vi "CPU_IRQ_handle.vi"(11 "registers":T1 {"P" format="%08b"; "PC" format="%04x"; "SP" format="%02x"; "Y" format="%02x"; "X" format="%02x"; "A" format="%02x"}) -> (3 "registers":T1 {"P" format="%08b"; "PC" format="%04x"; "SP" format="%02x"; "Y" format="%02x"; "X" format="%02x"; "A" format="%02x"})   [LabVIEW 2018]
uses:
  CPU_registers.ctl
  memory/CPU_MEM_Char_ROM_RE.vi
  CIA/CIA1/CIA1_glb.vi
  VIC/VIC_glb.vi
  memory/CPU_MEM_RAM.vi
  CPU_Port.vi
  memory/CPU_MEM_RAM_RE.vi
  memory/CPU_MEM_Basic_ROM_RE.vi
  memory/CPU_MEM_references.vi
  memory/CPU_MEM_VIC-II.vi
  memory/CPU_MEM_SID_RE.vi
  memory/CPU_MEM_Color_RE.vi
  memory/CPU_MEM_CIA 1.vi
  memory/CPU_MEM_CIA 2.vi
  memory/CPU_MEM_Kernal_ROM_RE.vi
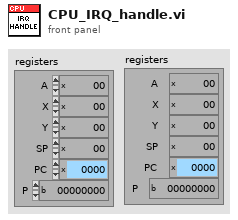
[diagram p1: front panel]
types:
  T1 = typedef "CPU_registers.ctl" = cluster{"A":u8, "X":u8, "Y":u8, "SP":u8, "PC":u16, "P":u8}
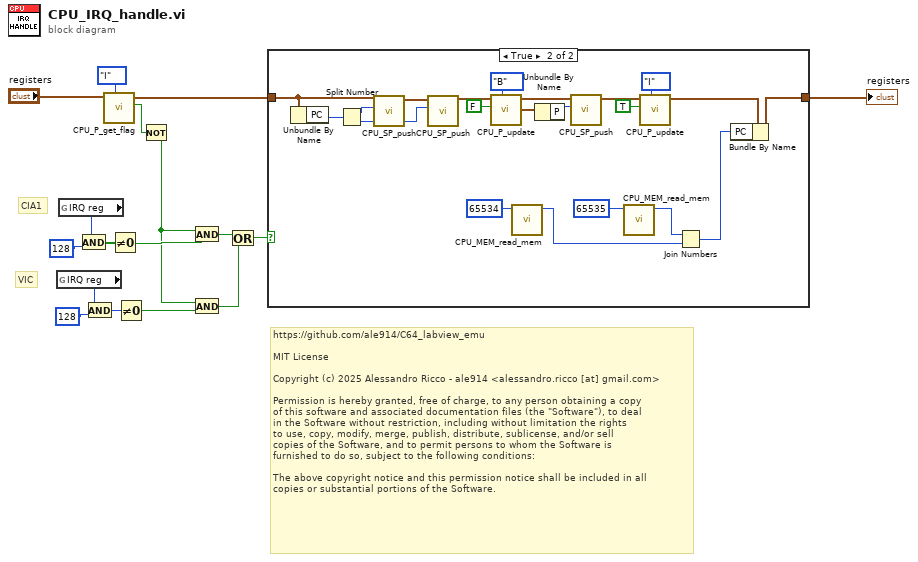
[diagram p0: block diagram]
diagram:
  # "https://github.com/ale914/C64_labview_emu\n\nMIT License\n\nCopyright (c) 2025 Alessandro Ricco - ale914 <alessandro.ricco [at] gmail.com>\n\nPermission is hereby granted, free of charge, to any person obtaining a copy\nof this software and associated documentation files (the \"Software\"), to deal\nin the Software without restriction, including without limitation the rights\nto use, copy, modify, merge, publish, distribute, sublicense, and/or sell\ncopies of the Software, and to permit persons to whom the Software is\nfurnished to do so, subject to the following conditions:\n\nThe above copyright notice and this permission notice shall be included in all\ncopies or substantial portions of the Software."
  # "VIC"
  # "CIA1"
  n1 = global read "VIC_glb.vi" "IRQ reg"() -> (w2:u8)
  n2 = global read "CIA1_glb.vi" "IRQ reg"() -> (w5:u8)
  n3 = And(x=w5, y=u8 128) -> (x .and. y?=w6:u8)
  n4 = And(x=w2, y=u8 128) -> (x .and. y?=w4:u8)
  n5 = call "CPU_P_get_flag.vi"("flag"=enum8{"C", "Z", "I", "D", "B", "V", "N"}."I", "registers"="registers") -> ("Value"=w12:bool, "registers"=w14:T1)  [unwired: 8 in]
  n6 = Not Equal To 0?(x=w6) -> (x != 0?=w11:bool)
  n7 = Not Equal To 0?(x=w4) -> (x != 0?=w1:bool)
  n8 = Not(x=w12) -> (.not. x?=w10:bool)
  n9 = And(x=w10, y=w11) -> (x .and. y?=w13:bool)
  n10 = And(x=w10, y=w1) -> (x .and. y?=w8:bool)
  n11 = Or(x=w13, y=w8) -> (x .or. y?=w9:bool)
  n12 = case shown="True" w9 {
    tunnel: w14 -> [w18 w33]
    tunnel: [w18 w20] -> w17
    frame False {
    }
    frame True {
      n13 = Unbundle By Name(w33) -> ("PC"=w38:u16)
      n14 = Split Number(x=w38) -> (hi(x)=w37:u8, lo(x)=w35:u8)
      n15 = call "CPU_SP_push.vi"("value"=w37, "registers"=w33) -> ("registers"=w36:T1)  [unwired: 9 in]
      n16 = call "CPU_SP_push.vi"("value"=w35, "registers"=w36) -> ("registers"=w30:T1)  [unwired: 9 in]
      n17 = call "CPU_P_update.vi"("flag"=enum8{"C", "Z", "I", "D", "B", "V", "N"}."B", "Value"=FALSE, "registers"=w30) -> ("registers"=w29:T1)  [unwired: 8 in]
      n18 = call "CPU_MEM_read_mem.vi"("address"=u16 65534) -> ("value out"=w25:u8)  [unwired: 10 in]
      n19 = Unbundle By Name(w29) -> ("P"=w31:u8)
      n20 = call "CPU_SP_push.vi"("value"=w31, "registers"=w29) -> ("registers"=w26:T1)  [unwired: 9 in]
      n21 = call "CPU_MEM_read_mem.vi"("address"=u16 65535) -> ("value out"=w24:u8)  [unwired: 10 in]
      n22 = call "CPU_P_update.vi"("flag"=enum8{"C", "Z", "I", "D", "B", "V", "N"}."I", "Value"=TRUE, "registers"=w26) -> ("registers"=w21:T1)  [unwired: 8 in]
      n23 = Join Numbers(hi=w24, lo=w25) -> ((hi.lo)=w19:u16)
      n24 = Bundle By Name(cluster=w21, "PC"=w19) -> (w20:T1)
    }
  }
  "registers" <- w17
